vi "macro_HolDrvController_Execute.vi"() -> ()   [LabVIEW 2019, in "Trajectory_Library.lvlib"]
uses:
  Trajectory_Library.lvlib
  TypeDef/POSE2D.ctl
  TypeDef/TRANSLATION2D.ctl
  TypeDef/ROTATION2D.ctl
  TypeDef/TRAJ_STATE.ctl
  ProfiledPIDController_NewPeriod.vi
  ProfiledPIDController_SetIntegratorRange.vi
  ProfiledPIDController_DisableContInput.vi
  ProfiledPIDController_EnableContInput.vi
  TrapProfConstraint_New.vi
  HolDrvCtrl_New.vi
  HolDrvCtrl_PackPID.vi
  HolDrvCtrl_SetTolerance.vi
  HolDrvCtrl_SetEnabled.vi
  HolDrvCtrl_Calculate_Trajectory.vi
  HolDrvCtrl_AtReference.vi
  TrapProfState_New.vi
  PIDController_NewPeriod.vi
  <vilib>/Rock Robotics/SystemInterfaces/NetworkCommunication/NetComm_UsageReport_report.vi
  PIDController_SetIntegratorRange.vi
  PIDController_DisableContinousInput.vi
  PIDController_EnableContinousInput.vi
  Conv_Deg_Radians.vi
  PIDController_Reset.vi
  HolDrvCtrl_Calculate.vi
  Pose2d_getXYAngle.vi
  Rotation2d_GetRadians.vi
  Rotation2d_GetAngleCosSin.vi
  Pose2d_RelativeTo.vi
  Pose2d_getRotation.vi
  Rotation2d_Minus.vi
  ProfiledPIDController_Calculate_Meas_Goal.vi
  PIDController_Calculate_SP_PV.vi
  ProfiledPIDController_Reset_PosOnly.vi
  ChassisSpeeds_FromFieldRelativeSpeeds.vi
  Transform2d_Create_PosePose.vi
  Pose2d_New_TRRO.vi
  Rotation2d_UnaryMinus.vi
  Rotation2d_RotateBy.vi
  ProfiledPIDController_SetGoal_PosOnly.vi
  ProfiledPIDController_Calculate_Meas.vi
  PIDController_SetSetpoint.vi
  PIDController_Calculate_PV.vi
  ProfiledPIDController_Reset.vi
  Rotation2d_GetCos.vi
  Rotation2d_GetSin.vi
  ChassisSpeeds_New.vi
  Translation2d_RotateBy.vi
  Translation2d_Minus.vi
  Rotation2d_CreateAngle.vi
  Rotation2d_CreateXY.vi
  ProfiledPIDController_SetGoal.vi
  TrapProfile_New.vi
  ProfiledPIDController_GetPeriod.vi
  TrapProfile_Calculate.vi
  ControllerUtil_GetModulusError.vi
  Translation2d_Create.vi
  Util_CalcDist.vi
  TrapProfile_ShouldFlipAcceleration.vi
  TrapProfile_Direct.vi
  PIDController_GetPeriod.vi
  Globals/Util_LibraryGlobals.vi
panel:
  in  "angleRef":T1={"VALUE"=0.0, "COS"=1.0, "SIN"=0.0} {"SIN" format="%13.4f"; "COS" format="%13.4f"; "VALUE" format="%13.4f"}
  in  "desiredTrajState":T2={"TimeSeconds"=0.0, "Velocity"=0.0, "Acceleration"=0.0, "POSE"={"TRANSLATION"={"X"=0.0, "Y"=0.0}, "ROTATION"={"VALUE"=0.0, "COS"=1.0, "SIN"=0.0}}, "Curvature"=0.0} {"POSE"."ROTATION"."SIN" format="%13.4f"; "POSE"."ROTATION"."COS" format="%13.4f"; "POSE"."ROTATION"."VALUE" format="%13.4f"; "POSE"."TRANSLATION"."Y" format="%14.3f"; "POSE"."TRANSLATION"."X" format="%14.3f"}
  in  "currentPose":T3={"TRANSLATION"={"X"=0.0, "Y"=0.0}, "ROTATION"={"VALUE"=0.0, "COS"=1.0, "SIN"=0.0}} {"ROTATION"."SIN" format="%13.4f"; "ROTATION"."COS" format="%13.4f"; "ROTATION"."VALUE" format="%13.4f"; "TRANSLATION"."Y" format="%14.3f"; "TRANSLATION"."X" format="%14.3f"}
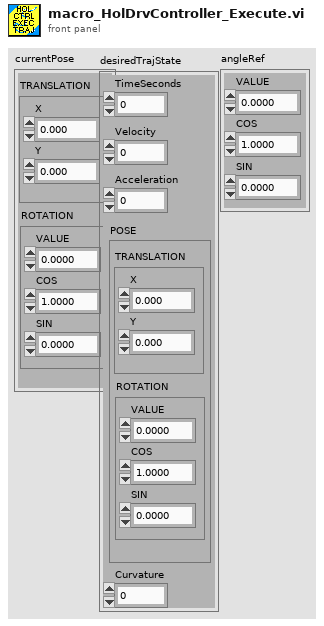
[diagram p1: front panel]
types:
  T1 = typedef "Trajectory_Library.lvlib/ROTATION2D.ctl" = cluster{"VALUE":dbl, "COS":dbl, "SIN":dbl}
  T2 = typedef "Trajectory_Library.lvlib/TRAJ_STATE.ctl" = cluster{"TimeSeconds":dbl, "Velocity":dbl, "Acceleration":dbl, "POSE":T3, "Curvature":dbl}
  T3 = typedef "Trajectory_Library.lvlib/POSE2D.ctl" = cluster{"TRANSLATION":T4, "ROTATION":T1}
  T4 = typedef "Trajectory_Library.lvlib/TRANSLATION2D.ctl" = cluster{"X":dbl, "Y":dbl}
  T5 = typedef "Trajectory_Library.lvlib/PID_TUNING.ctl" = cluster{"Kp":dbl, "Ki":dbl, "Kd":dbl, "MaximumIntegral":dbl, "MinimumIntegral":dbl, "IntegralZone":dbl}
  T6 = typedef "Trajectory_Library.lvlib/PROFILED_PID_CONTROLLER.ctl" = cluster{"Controller":T7, "Goal":T8, "Setpoint":T8, "Constraint":T9}
  T7 = typedef "Trajectory_Library.lvlib/PID_CONTROLLER.ctl" = cluster{"Kp":dbl, "Ki":dbl, "Kd":dbl, "Period":dbl, "Max_Integral":dbl, "Min_Integral":dbl, "Max_Input":dbl, "Min_Input":dbl, "Continuous":bool, "PositionError":dbl, "VelocityError":dbl, "PrevError":dbl, "Total_Integral":dbl, "PositionTolerance":dbl, "VelocityTolerance":dbl, "SetPoint":dbl, "Kf":dbl, "Prev_Deriv":dbl, "Prev_Deriv 2":dbl, "DerivativeFilter":bool, "Min_Output":dbl, "Max_Output":dbl, "Prev_F_P":dbl, "Prev_F_P_2":dbl, "AntiWindupActive":bool, "Measurement":dbl, "IntegralZone":dbl}
  T8 = typedef "Trajectory_Library.lvlib/TRAPEZOID_PROFILE_STATE.ctl" = cluster{"Position":dbl, "Velocity":dbl}
  T9 = typedef "Trajectory_Library.lvlib/TRAPEZOID_PROFILE_CONSTRAINT.ctl" = cluster{"MaxVelocity":dbl, "MaxAcceleration":dbl}
  T10 = typedef "Trajectory_Library.lvlib/HOLONOMIC_PACK_TUNING.ctl" = cluster{"X PID Tuning":T5, "Y PID Tuning":T5, "thetaProfiledPID_CTRL":T6}
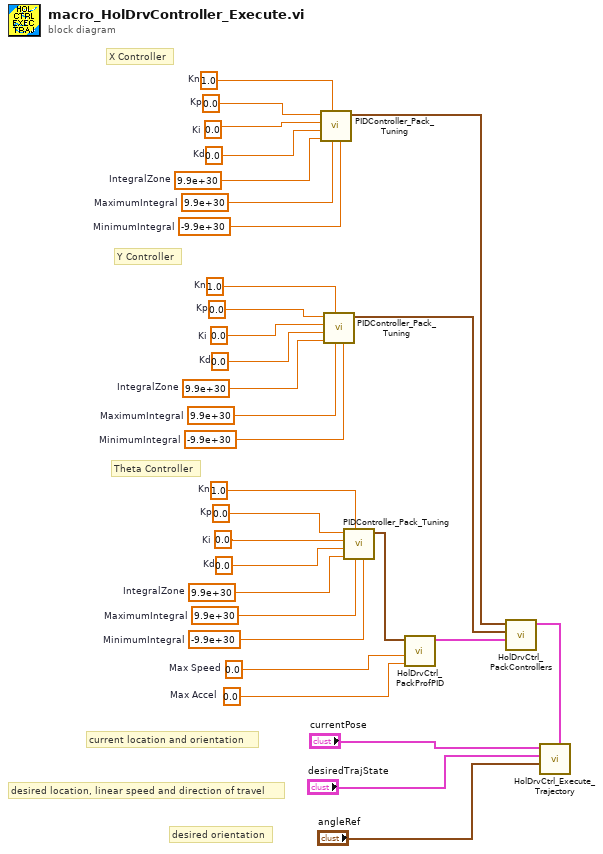
[diagram p0: block diagram]
diagram:
  w1 = 9.9e+30  # IntegralZone
  w2 = 9.9e+30  # IntegralZone
  w3 = 9.9e+30  # IntegralZone
  w26 = 1.0  # Kn
  w23 = 0.0  # Kp
  w14 = 0.0  # Ki
  w13 = 0.0  # Kd
  w12 = 9.9e+30  # MaximumIntegral
  w11 = -9.9e+30  # MinimumIntegral
  w28 = 1.0  # Kn
  w25 = 0.0  # Kp
  w22 = 0.0  # Ki
  w21 = 0.0  # Kd
  w20 = 9.9e+30  # MaximumIntegral
  w19 = -9.9e+30  # MinimumIntegral
  w27 = 1.0  # Kn
  w24 = 0.0  # Kp
  w18 = 0.0  # Ki
  w17 = 0.0  # Kd
  w16 = 9.9e+30  # MaximumIntegral
  w15 = -9.9e+30  # MinimumIntegral
  w29 = 0.0  # Max Accel
  w30 = 0.0  # Max Speed
  # "desired orientation"
  # "desired location, linear speed and direction of travel"
  # "current location and orientation"
  # "Theta Controller"
  # "Y Controller"
  # "X Controller"
  n1 = call "PIDController_Pack_Tuning.vi"("MinimumIntegral"=w19, "MaximumIntegral"=w20, "Kn"=w28, "IntegralZone"=w3, "Kd"=w21, "Ki"=w22, "Kp"=w25) -> ("PID Tuning"=w10:T5)  [unwired: 4 in]
  n2 = call "PIDController_Pack_Tuning.vi"("MinimumIntegral"=w15, "MaximumIntegral"=w16, "Kn"=w27, "IntegralZone"=w2, "Kd"=w17, "Ki"=w18, "Kp"=w24) -> ("PID Tuning"=w9:T5)  [unwired: 4 in]
  n3 = call "PIDController_Pack_Tuning.vi"("MinimumIntegral"=w11, "MaximumIntegral"=w12, "Kn"=w26, "IntegralZone"=w1, "Kd"=w13, "Ki"=w14, "Kp"=w23) -> ("PID Tuning"=w31:T5)  [unwired: 4 in]
  n4 = call "HolDrvCtrl_PackProfPID.vi"("Max Accel"=w29, "Max Speed"=w30, "Theta PID Tuning"=w31) -> ("Theta PID CONTROLLER"=w8:T6)  [unwired: 8 in]
  n5 = call "HolDrvCtrl_PackControllers.vi"("thetaProfiledPID_CTRL"=w8, "Y PID Tuning"=w9, "X PID Tuning"=w10) -> ("HOLONOMIC_CTRL_PACK_TUNING"=w7:T10)  [unwired: 8 in]
  n6 = call "HolDrvCtrl_Execute_Trajectory.vi"("HOLONOMIC_CTRL_PACK_TUNING"=w7, "angleRef"="angleRef", "desiredTrajState"="desiredTrajState", "currentPose"="currentPose") -> ()  [unwired: 5 in, 3 out]
